vi "Read Request Context.vi"(8 "error in":errorcluster) -> (0 "error out":errorcluster, 2 "found?":bool, 3 "context":string)   [LabVIEW 2020, in "MCP Server.lvlib"]
doc: "Reads the request context of the tools/call that is running: the element of the named queue \"MCP Request Context\", written by Handle MCP Request.vi. The queue is only looked up, never created, and the element stays in the queue.\n\nfound? is FALSE outside a request; context is then empty. Used by Ask User.vi and Get Request Stream.vi.\n\nRuns regardless of error in, which is passed through unchanged; queue errors only make found? FALSE."
uses:
  MCP Server.lvlib
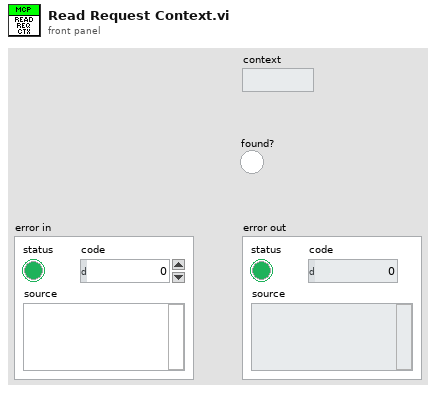
[diagram p1: front panel]
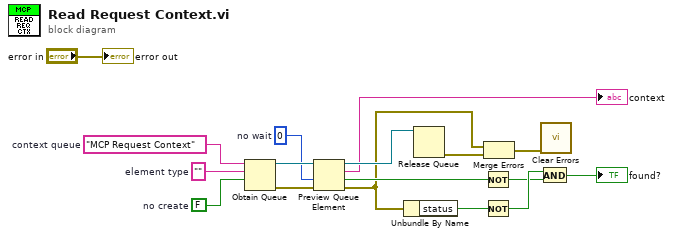
[diagram p0: block diagram]
diagram:
  w13 = 0  # no wait
  w15 = FALSE  # no create
  w16 = ""  # element type
  w17 = "MCP Request Context"  # context queue
  n1 = Obtain Queue(name (unnamed)=w17, element data type=w16, create if not found? (T)=w15) -> (queue out=w14:refnum<queue>, error out=w12:errorcluster)  [unwired: 2 in, 1 out]
  n2 = Preview Queue Element(queue=w14, timeout in ms (-1)=w13, error in (no error)=w12) -> (queue out=w11:refnum<queue>, element=→"context":string, timed out?=w9:bool, error out=w6:errorcluster)
  n3 = Unbundle By Name(w6) -> ("status"=w10:bool)
  n4 = Release Queue(queue=w11) -> (error out=w5:errorcluster)  [unwired: 2 in, 2 out]
  n5 = Not(x=w9) -> (.not. x?=w7:bool)
  n6 = Not(x=w10) -> (.not. x?=w8:bool)
  n7 = Merge Errors(w6, w5) -> (w4:errorcluster)
  n8 = And(x=w8, y=w7) -> (x .and. y?=→"found?":bool)
  n9 = call <vilib>:"Clear Errors.vi"("error in (no error)"=w4) -> ()  [unwired: 5 in, 2 out]
  "error out" <- "error in"
